vi "Frame Order 2.vi"() -> ()   [LabVIEW 2026]
doc: "Probe two: nested case in the visible frame, and a second top-level case."
panel:
  in  "s3":string="m"
  in  "s2":string="p"
  in  "s1":string="A"
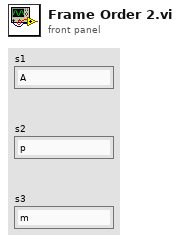
[diagram p1: front panel]
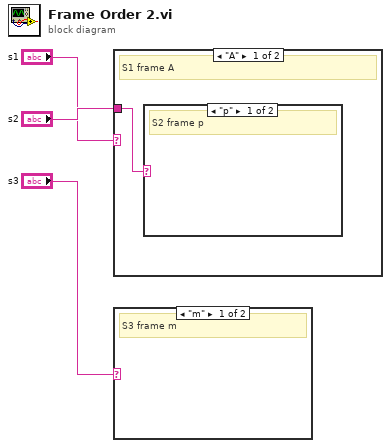
[diagram p0: block diagram]
diagram:
  n1 = case shown="\"b\", Default" "s1" {
    tunnel: "s2" -> [w4 _]
    frame "A" {
      # "S1 frame A"
      n2 = case shown="\"b\", Default" w4 {
        frame "p" {
          # "S2 frame p"
        }
        frame Default {
          # "S2 frame q"
        }
      }
    }
    frame Default {
      # "S1 frame B"
    }
  }
  n3 = case shown="\"b\", Default" "s3" {
    frame "m" {
      # "S3 frame m"
    }
    frame Default {
      # "S3 frame n"
    }
  }
